vi "Execute with Default Process Model.vi"() -> ()   [LabVIEW 2020]
uses:
  TSnax/Execution/Set Entry Sequence.vi
  TSnax/Execution/Set SequenceFile.vi
  TSnax/Execution/Get Result Status.vi
  TSnax/Engine/Engine.lvclass
  TSnax/Execution/Execution.lvclass
  TSnax/SequenceFile/SequenceFile.lvclass
panel:
  in  "Entry Point":string="Single Pass"
  out "Status":string
  in  "SequenceFile Path":path=path "C:/Users/Public/Documents/National Instruments/TestStand 2020 (32-bit)/Examples/Demos/Computer Motherboard Test/LabVIEW/Computer Motherboard Test Sequence.seq"
  # "1."
  # "2."
  # "1. Select the sequence file you'd like to run.\n\n2. Enter the name of the entry point to use in the process model. This is usually 'Test UUTs' or 'Single Pass' for models that ship with TestStand."
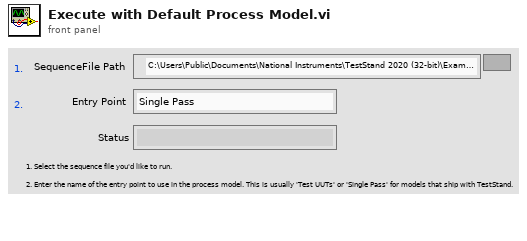
[diagram p1: front panel]
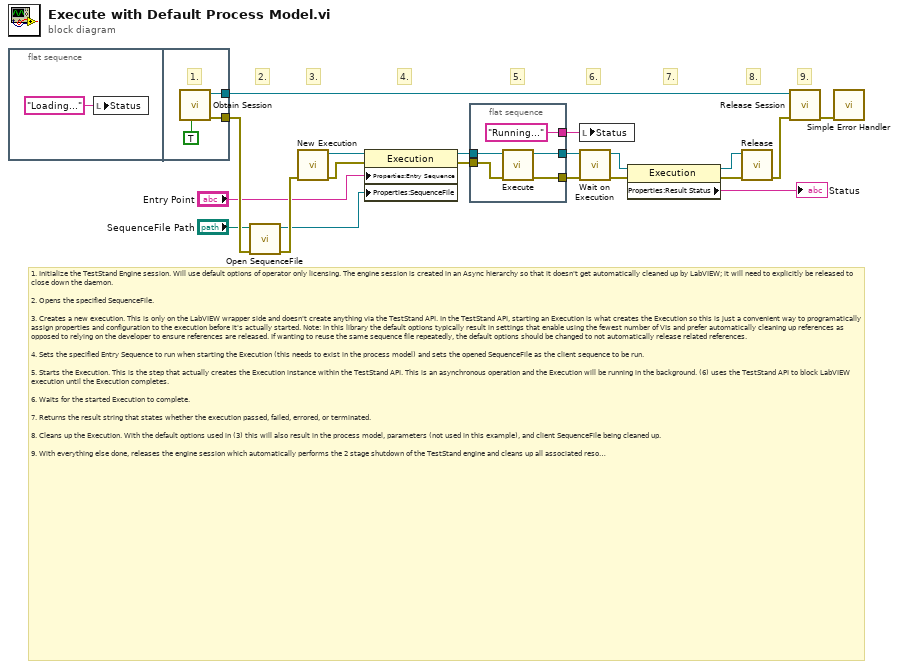
[diagram p0: block diagram]
diagram:
  # "1. Initialize the TestStand Engine session. Will use default options of operator only licensing. The engine session is created in an Async hierarchy so that it doesn't get automatically cleaned up by LabVIEW; it will need to explicitly be released to close down the daemon.\n\n2. Opens the specified SequenceFile. \n\n3. Creates a new execution. This is only on the LabVIEW wrapper side and doesn't create anything via the TestStand API. In the TestStand API, starting an Execution is what creates the Execution so this is just a convenient way to programatically assign properties and configuration to the execution before it's actually started. Note: In this library the default options typically result in settings that enable using the fewest number of VIs and prefer automatically cleaning up references as opposed to relying on the developer to ensure references are released. If wanting to reuse the same sequence file repeatedly, the default options should be changed to not automatically release related references.\n\n4. Sets the specified Entry Sequence to run when starting the Execution (this needs to exist in the process model) and sets the opened SequenceFile as the client sequence to be run.\n\n5. Starts the Execution. This is the step that actually creates the Execution instance within the TestStand API. This is an asynchronous operation and the Execution will be running in the background. (6) uses the TestStand API to block LabVIEW execution until the Execution completes.\n\n6. Waits for the started Execution to complete.\n\n7. Returns the result string that states whether the execution passed, failed, errored, or terminated.\n\n8. Cleans up the Execution. With the default options used in (3) this will also result in the process model, parameters (not used in this example), and client SequenceFile being cleaned up.\n\n9. With everything else done, releases the engine session which automatically performs the 2 stage shutdown of the TestStand engine and cleans up all associated resources."
  # "9."
  # "8."
  # "7."
  # "6."
  # "5."
  # "4."
  # "3."
  # "2."
  n1 = flat-sequence {
    tunnel: [w24] -> w1
    tunnel: [w23] -> w19
    frame #0 {
      n2 = local write "Status"("Loading..." ("Status")) -> ()
    }
    frame #1 {
      # "1."
      n3 = call "Obtain Session.vi"("Debug Daemon (Dev Only)"=TRUE) -> ("error out"=w23:errorcluster, "Engine out"=w24:refnum<class "Engine.lvclass">)  [unwired: 9 in]
    }
  }
  n4 = call "Open SequenceFile.vi"("error in (no error)"=w19, "Path"="SequenceFile Path") -> ("error out"=w20:errorcluster, "SequenceFile out"=w2:refnum<class "SequenceFile.lvclass">)  [unwired: 8 in]
  n5 = call "New Execution.vi"("error in (no error)"=w20) -> ("error out"=w3:errorcluster, "Execution out"=w4:refnum<class "Execution.lvclass">)  [unwired: 9 in]
  n6 = property class="Execution"(reference=w4, error in=w3, "Properties:Entry Sequence"="Entry Point", "Properties:SequenceFile"=w2) -> (reference out=w17:refnum<class "Execution.lvclass">, error out=w16:errorcluster)
  n7 = flat-sequence {
    tunnel: w17 -> [w29]
    tunnel: w16 -> [w28]
    tunnel: ["Running..." ("Status")] -> w15
    tunnel: [w26] -> w14
    tunnel: [w25] -> w13
    frame #0 {
      n8 = call "Execute.vi"("error in (no error)"=w28, "Execution in"=w29) -> ("error out"=w25:errorcluster, "Execution out"=w26:refnum<class "Execution.lvclass">)  [unwired: 8 in]
    }
  }
  n9 = local write "Status"(w15) -> ()
  n10 = call "Wait on Execution.vi"("error in (no error)"=w13, "Execution in"=w14) -> ("error out"=w11:errorcluster, "Execution out"=w12:refnum<class "Execution.lvclass">)  [unwired: 7 in, 1 out]
  n11 = property class="Execution"(reference=w12, error in=w11) -> (reference out=w9:refnum<class "Execution.lvclass">, error out=w8:errorcluster, "Properties:Result Status"=→"Status":string)
  n12 = call-dynamic "Release.vi"("error in (no error)"=w8, "Execution in"=w9) -> ("error out"=w7:errorcluster)  [unwired: 9 in]
  n13 = call "Release Session.vi"("error in (no error)"=w7, "Engine in"=w1) -> ("error out"=w6:errorcluster)  [unwired: 9 in]
  n14 = call <vilib>:"Simple Error Handler.vi"("error in (no error)"=w6) -> ()  [unwired: 4 in, 5 out]
